vi "Extract All Files to Directory.vi"(8 "error in (no error)":errorcluster, 10 "Extract to Dir":path, 11 "Zip File Path":path) -> (0 "error out":errorcluster)   [LabVIEW 2020, in "Command-Line Zip.lvlib"]
uses:
  Command-Line Zip.lvlib
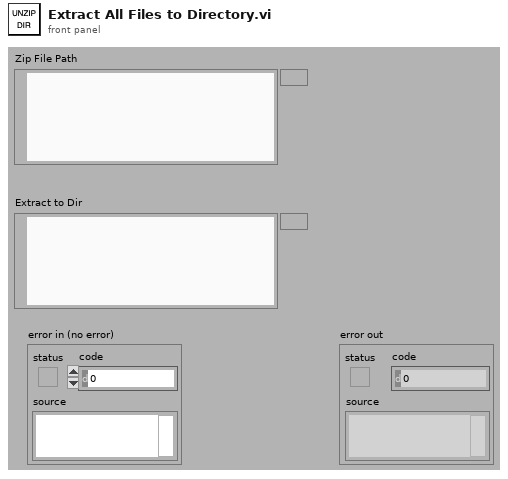
[diagram p1: front panel]
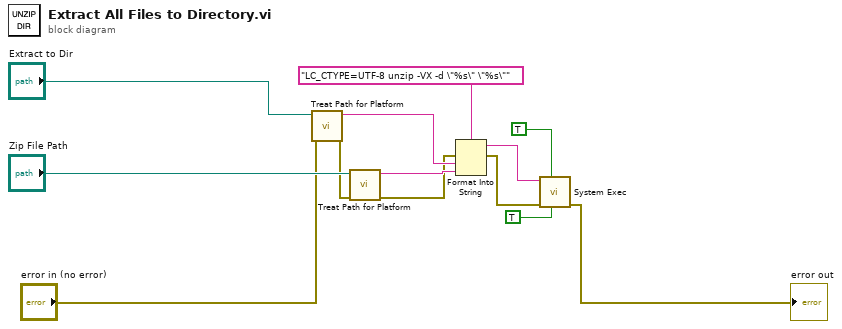
[diagram p0: block diagram]
diagram:
  n1 = call "Treat Path for Platform.vi"("error in (no error)"="error in (no error)", "File Path"="Extract to Dir") -> ("error out"=w6:errorcluster, "Path for CLI"=w7:string)  [unwired: 8 in]
  n2 = call "Treat Path for Platform.vi"("error in (no error)"=w6, "File Path"="Zip File Path") -> ("error out"=w5:errorcluster, "Path for CLI"=w8:string)  [unwired: 8 in]
  n3 = Format Into String(format string="LC_CTYPE=UTF-8 unzip -VX -d \"%s\" \"%s\"", error in=w5, w7, w8) -> (resulting string=w3:string, error out=w4:errorcluster)  [unwired: 1 in]
  n4 = call <vilib>:"System Exec.vi"("run minimized? (F)"=TRUE, "wait until completion? (T)"=TRUE, "error in (no error)"=w4, "command line"=w3) -> ("error out"=→"error out":errorcluster)  [unwired: 4 in, 3 out]
